vi "I2C An Out M5Stack8ChServo.vi"() -> ()   [LabVIEW 2020, in "CTI-Scratchpad.lvlib"]
uses:
  CTI-Scratchpad.lvlib
  CTI/Identity.ctl
  CTI/Error Reporting.ctl
  CTI-Peripheral/Analog Output/I2C PWM/M5Stack I2C 8Ch PWM/Private/registers.ctl
  CTI-Peripheral/Analog Output/I2C PWM/M5Stack I2C 8Ch PWM/Private/GPIOOperationModes.ctl
  CTI/I2C Address.ctl
  CTI/GPIO Number.ctl
  CTI/I2C Number.ctl
  CTI/Session/Session.lvclass
  CTI-Peripheral/Analog Output/I2C PWM/M5Stack I2C 8Ch PWM/M5Stack I2C 8Ch Servo.lvclass
  CTI/VisaComms/VisaComms.lvclass
  CTI/CTI.lvlib
panel:
  in  "CH7":u8(slide)=90 scale=0.0..180.0
  in  "CH6":u8(slide)=90 scale=0.0..180.0
  in  "CH5":u8(slide)=90 scale=0.0..180.0
  in  "CH4":u8(slide)=90 scale=0.0..180.0
  in  "CH3":u8(slide)=90 scale=0.0..180.0
  in  "CH2":u8(slide)=90 scale=0.0..180.0
  in  "CH1":u8(slide)=90 scale=0.0..180.0
  in  "CH0":u8(slide)=90 scale=0.0..180.0
  out "loop":i32
  in  "stop":bool
  out "Identity":T1
  in  "Grove Connector":enum16{"I2C0", "I2C1"}(ring)
  out "error out":errorcluster
  in  "Port":refnum<visa-resource-name>="COM4"
  # "https://shop.m5stack.com/products/8-channel-servo-driver-unit-stm32f030?srsltid=AYCX9vJPlmHf0PEe2hkOf9JoORrCSCLFPOOBXTb4mmNWhcA5r_nAQ2T2"
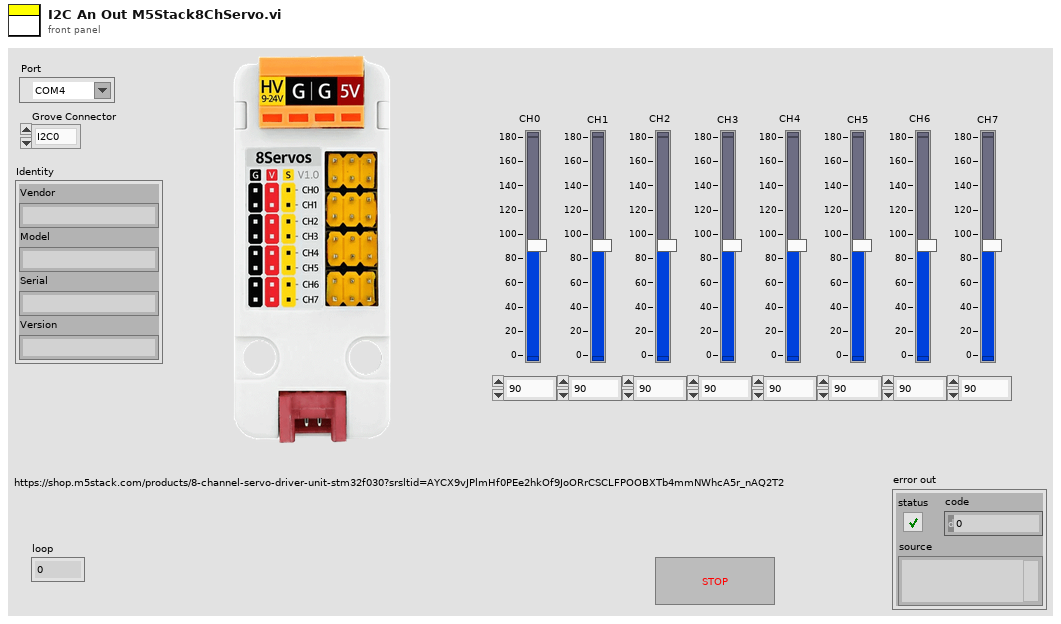
[diagram p1: front panel]
types:
  T1 = typedef "CTI.lvlib/Identity.ctl" = cluster{"Vendor":string, "Model":string, "Serial":string, "Version":string}
  T2 = typedef "CTI.lvlib/I2C Address.ctl" = u8
  T3 = typedef "CTI-Peripheral.lvlib/M5Stack I2C 8Ch Servo.lvclass/GPIOOperationModes.ctl" = u16
  T4 = typedef "CTI-Peripheral.lvlib/M5Stack I2C 8Ch Servo.lvclass/registers.ctl" = u8
  T5 = typedef "CTI.lvlib/Error Reporting.ctl" = enum16{"Minimal", "Moderate", "Full"}
  T6 = typedef "CTI.lvlib/I2C Number.ctl" = i8
  T7 = typedef "CTI.lvlib/GPIO Number.ctl" = i8
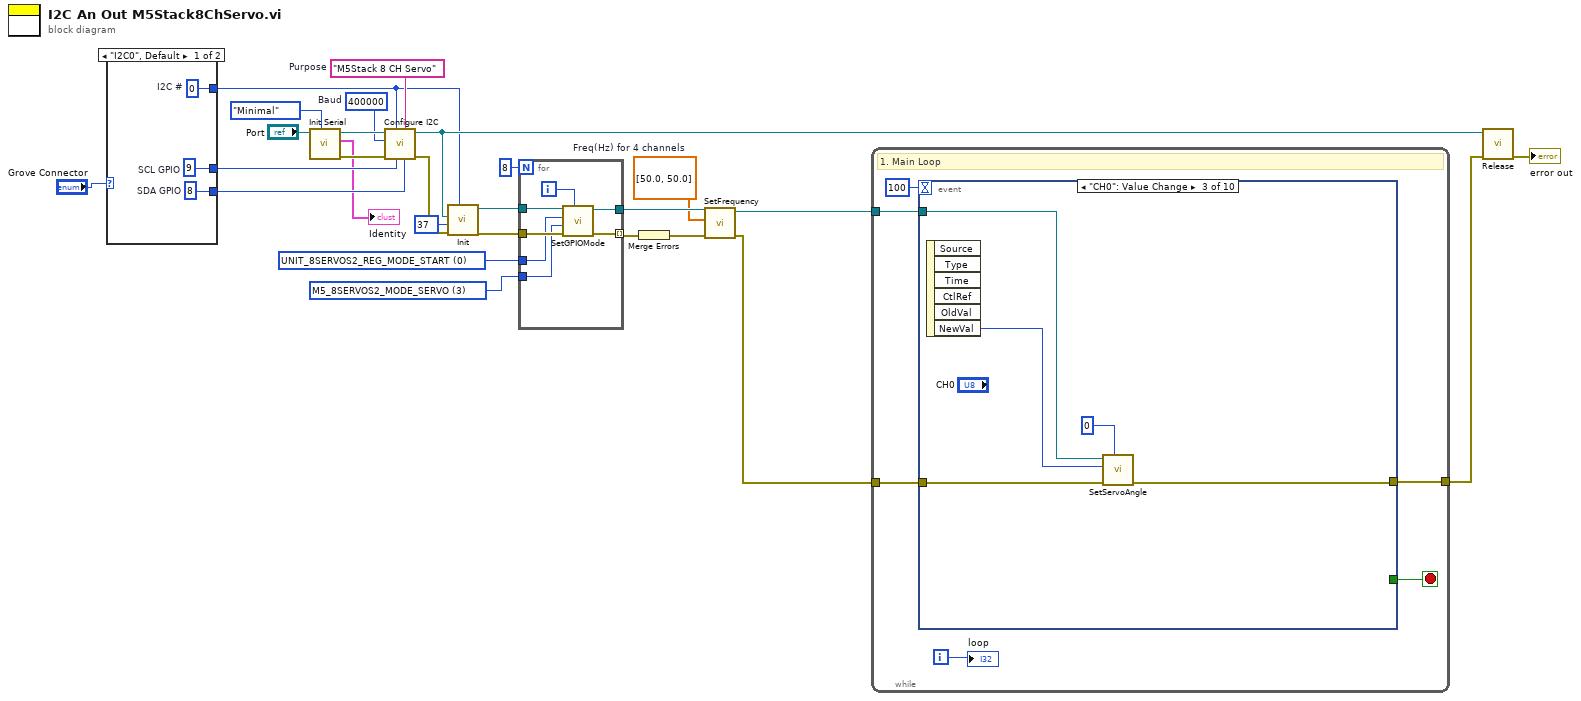
[diagram p0: block diagram]
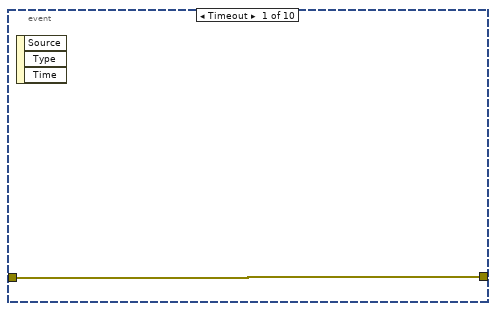
[diagram p2: hidden frame]
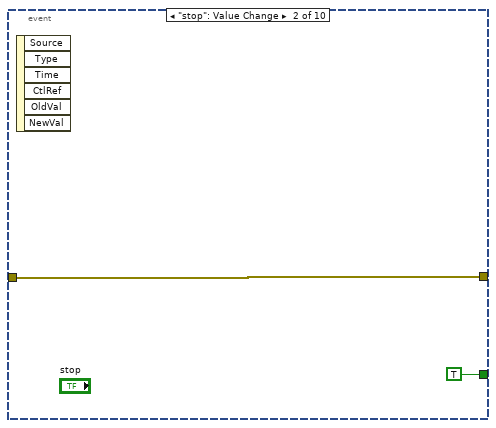
[diagram p3: hidden frame]
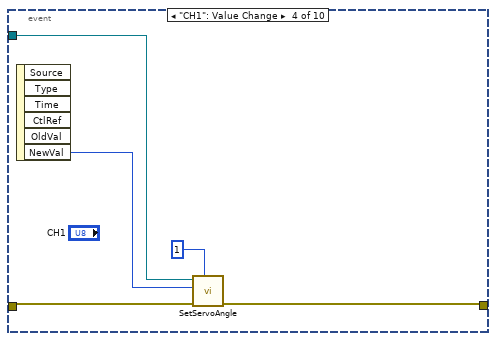
[diagram p4: hidden frame]
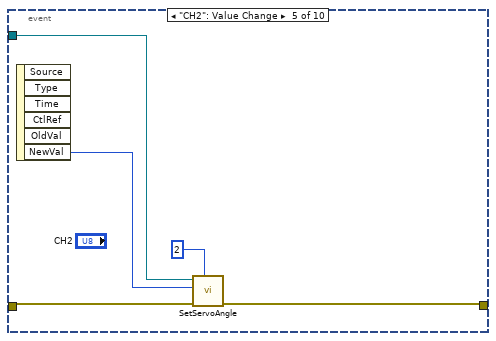
[diagram p5: hidden frame]
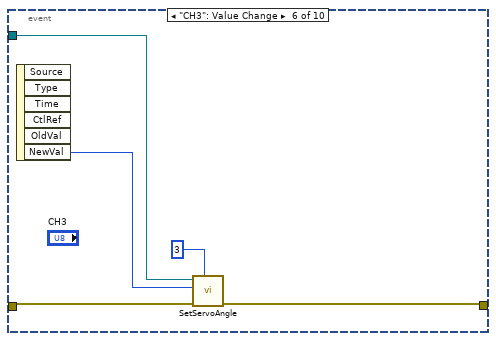
[diagram p6: hidden frame]
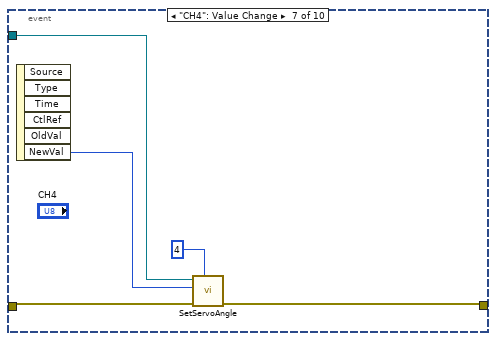
[diagram p7: hidden frame]
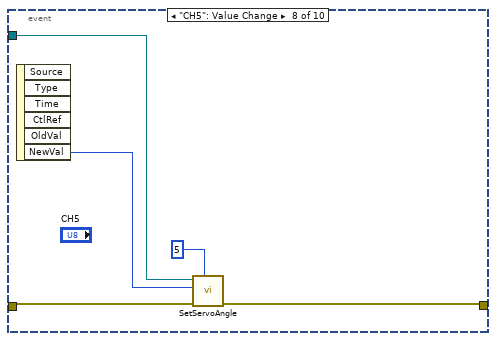
[diagram p8: hidden frame]
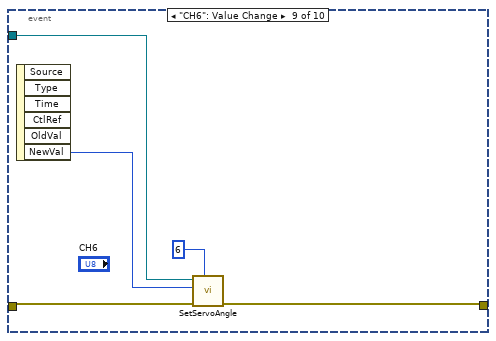
[diagram p9: hidden frame]
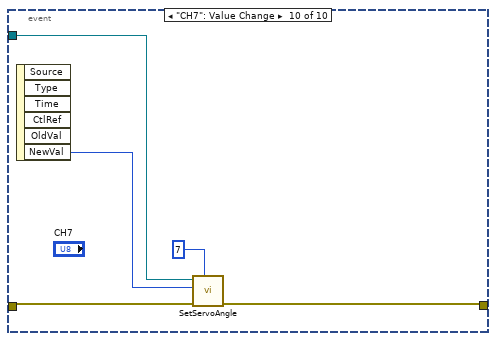
[diagram p10: hidden frame]
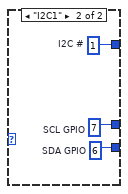
[diagram p11: hidden frame]
diagram:
  w4 = sgl[] [50.0, 50.0]  # Freq(Hz) for 4 channels
  w6 = T3 3 items=["M5_8SERVOS2_MODE_INPUT  ", "M5_8SERVOS2_MODE_OUTPUT ", "M5_8SERVOS2_MODE_ADC    ", "M5_8SERVOS2_MODE_SERVO  ", "M5_8SERVOS2_MODE_RGB    ", "M5_8SERVOS2_MODE_PWM    "] ("Op Mode")
  w7 = T4 0 items=["UNIT_8SERVOS2_REG_MODE_START"=0, "UNIT_8SERVOS2_REG_INPUT_PULL_START"=16, "UNIT_8SERVOS2_REG_INPUT_STATUS_START"=32, "UNIT_8SERVOS2_REG_OUTPUT_STATUS_START"=48, "UNIT_8SERVOS2_REG_ADC_START"=64, "UNIT_8SERVOS2_REG_SERVO_START"=80, "UNIT_8SERVOS2_REG_RGB_CONF_START"=96, "UNIT_8SERVOS2_REG_PWM_DUTY_START"=112, "UNIT_8SERVOS2_REG_RGB_BUFFER_START"=128, "UNIT_8SERVOS2_REG_TIM_FREQ_START"=208, "UNIT_8SERVOS2_REG_UID_START"=224, "UNIT_8SERVOS2_REG_UID_END"=235, "UNIT_8SERVOS2_REG_SYS_ANALOG_START"=240, "UNIT_8SERVOS2_REG_ADDR_OFFSET"=248, "UNIT_8SERVOS2_REG_I2C_ADDR_REFRESH"=252, "UNIT_8SERVOS2_REG_VERSION"=254, "UNIT_8SERVOS2_REG_I2C_ADDR"=255] ("Registers")
  w22 = "M5Stack 8 CH Servo"  # Purpose
  w23 = u32 400000  # Baud
  n1 = case shown="\"I2C0\", Default" "Grove Connector" {
    tunnel: [w30 w33] -> w20
    tunnel: [w29 w32] -> w19
    tunnel: [w28 w31] -> w13
    frame "I2C0", Default {
      w28 = T6 0  # I2C #
      w29 = T7 8  # SDA GPIO
      w30 = T7 9  # SCL GPIO
    }
    frame "I2C1" {
      w31 = T6 1  # I2C #
      w32 = T7 6  # SDA GPIO
      w33 = T7 7  # SCL GPIO
    }
  }
  n2 = call "Init Serial.vi"("Error Checking (Full)"=Error_Reporting."Minimal", "VISA resource name in"="Port") -> ("error out"=w24:errorcluster, "Identity"=→"Identity":T1, "Session"=w25:refnum<class "Session.lvclass">)  [unwired: 7 in]
  n3 = call "Configure I2C.vi"("SDA GPIO"=w19, "Purpose (\"I2C\")"=w22, "SCL GPIO"=w20, "I2C #"=w13, "error in (no error)"=w24, "Baud"=w23, "Session in"=w25) -> ("error out"=w14:errorcluster, "Session out"=w15:refnum<class "Session.lvclass">)  [unwired: 3 in]
  n4 = call "Init.vi"("I2C #"=w13, "error in (no error)"=w14, "Address"=T2 37, "Session In"=w15) -> ("error out"=w10:errorcluster, "M5Stack8ChPWM Out"=w12:refnum<class "M5Stack I2C 8Ch Servo.lvclass">)  [unwired: 6 in]
  n5 = for {
    N: 8 -> [_]
    tunnel: w12 -> [w40]
    tunnel: w10 -> [w38]
    tunnel: [w37] -> w9 mode=indexing
    tunnel: w7 -> [w36]
    tunnel: w6 -> [w35]
    tunnel: [w34] -> w5
    i -> [w39]
    n6 = call-dynamic "SetGPIOMode.vi"("Channel"=w39, "error in (no error)"=w38, "Op Mode"=w35, "Registers"=w36, "M5Stack I2C 8Ch Servo in"=w40) -> ("error out"=w37:errorcluster, "M5Stack I2C 8Ch Servo out"=w34:refnum<class "M5Stack I2C 8Ch Servo.lvclass">)  [unwired: 5 in]
  }
  n7 = Merge Errors(w9) -> (w8:errorcluster)
  n8 = call-dynamic "SetFrequency.vi"("error in (no error)"=w8, "Freq"=w4, "M5Stack I2C 8Ch Servo in"=w5) -> ("error out"=w1:errorcluster, "M5Stack I2C 8Ch Servo out"=w2:refnum<class "M5Stack I2C 8Ch Servo.lvclass">)  [unwired: 7 in]
  n9 = while {
    tunnel: w1 -> [w45]
    tunnel: w2 -> [w46]
    tunnel: [w43] -> w17
    i -> [w44]
    stop <- w42 stop-if-true
    # "1. Main Loop"
    n10 = event shown="[2] \"CH0\": Value Change" {
      selector: _ -> [_ _ _ _ _ _ _ _ _ _]
      dyn-events: _ -> [_ _ _ _ _ _ _ _ _ _]
      timeout: 100 -> [_ _ _ _ _ _ _ _ _ _]
      tunnel: w46 -> [_ _ w53 w57 w62 w67 w72 w77 w82 w87]
      tunnel: w45 -> [w47 w48 w54 w59 w64 w69 w74 w79 w84 w89]
      tunnel: [w47 w48 w50 w58 w63 w68 w73 w78 w83 w88] -> w43
      tunnel: [_ TRUE _ _ _ _ _ _ _ _] -> w42
      event Timeout {
        n11 = event-data() -> ()  [unwired: 1 in, 3 out]
      }
      event "stop": Value Change {
        n12 = event-data() -> ()  [unwired: 1 in, 6 out]
      }
      event "CH0": Value Change {
        n13 = event-data() -> ("NewVal"=w52:u8)  [unwired: 1 in, 5 out]
        n14 = call-dynamic "SetServoAngle.vi"("Channel"=u8 0, "error in (no error)"=w54, "Angle"=w52, "M5Stack I2C 8Ch Servo in"=w53) -> ("error out"=w50:errorcluster)  [unwired: 6 in, 1 out]
      }
      event "CH1": Value Change {
        n15 = event-data() -> ("NewVal"=w56:u8)  [unwired: 1 in, 5 out]
        n16 = call-dynamic "SetServoAngle.vi"("Channel"=u8 1, "error in (no error)"=w59, "Angle"=w56, "M5Stack I2C 8Ch Servo in"=w57) -> ("error out"=w58:errorcluster)  [unwired: 6 in, 1 out]
      }
      event "CH2": Value Change {
        n17 = event-data() -> ("NewVal"=w61:u8)  [unwired: 1 in, 5 out]
        n18 = call-dynamic "SetServoAngle.vi"("Channel"=u8 2, "error in (no error)"=w64, "Angle"=w61, "M5Stack I2C 8Ch Servo in"=w62) -> ("error out"=w63:errorcluster)  [unwired: 6 in, 1 out]
      }
      event "CH3": Value Change {
        n19 = event-data() -> ("NewVal"=w66:u8)  [unwired: 1 in, 5 out]
        n20 = call-dynamic "SetServoAngle.vi"("Channel"=u8 3, "error in (no error)"=w69, "Angle"=w66, "M5Stack I2C 8Ch Servo in"=w67) -> ("error out"=w68:errorcluster)  [unwired: 6 in, 1 out]
      }
      event "CH4": Value Change {
        n21 = event-data() -> ("NewVal"=w71:u8)  [unwired: 1 in, 5 out]
        n22 = call-dynamic "SetServoAngle.vi"("Channel"=u8 4, "error in (no error)"=w74, "Angle"=w71, "M5Stack I2C 8Ch Servo in"=w72) -> ("error out"=w73:errorcluster)  [unwired: 6 in, 1 out]
      }
      event "CH5": Value Change {
        n23 = event-data() -> ("NewVal"=w76:u8)  [unwired: 1 in, 5 out]
        n24 = call-dynamic "SetServoAngle.vi"("Channel"=u8 5, "error in (no error)"=w79, "Angle"=w76, "M5Stack I2C 8Ch Servo in"=w77) -> ("error out"=w78:errorcluster)  [unwired: 6 in, 1 out]
      }
      event "CH6": Value Change {
        n25 = event-data() -> ("NewVal"=w81:u8)  [unwired: 1 in, 5 out]
        n26 = call-dynamic "SetServoAngle.vi"("Channel"=u8 6, "error in (no error)"=w84, "Angle"=w81, "M5Stack I2C 8Ch Servo in"=w82) -> ("error out"=w83:errorcluster)  [unwired: 6 in, 1 out]
      }
      event "CH7": Value Change {
        n27 = event-data() -> ("NewVal"=w86:u8)  [unwired: 1 in, 5 out]
        n28 = call-dynamic "SetServoAngle.vi"("Channel"=u8 7, "error in (no error)"=w89, "Angle"=w86, "M5Stack I2C 8Ch Servo in"=w87) -> ("error out"=w88:errorcluster)  [unwired: 6 in, 1 out]
      }
    }
    "loop" <- w44
  }
  n29 = call-dynamic "Release.vi"("error in (no error)"=w17, "Session in"=w15) -> ("error out"=→"error out":errorcluster)  [unwired: 9 in]
